vi "FT10xx系列_Coincidence_sample_1.0.3.vi"() -> ()   [LabVIEW 2017]
uses:
  National Instruments/LabVIEW 2017/user.lib/smncsftmt/smncsftmt.lvlib
panel:
  in  "通道选择":i32=1 min=1 max=8
  in  "C18 16":bool
  in  "C17 16":bool
  in  "C16 16":bool
  in  "C15 16":bool
  in  "C14 16":bool
  in  "C13 16":bool
  in  "C12 16":bool=TRUE
  in  "C11 16":bool=TRUE
  in  "窗口宽度(ns)":dbl=1000.0
  in  "停止":bool
  out "error out":errorcluster
  out "通道计数":u64
  out "符合计数":u32
  in  "统计时间(s)":dbl=1.0
  in  "保存路径":path=path "D:/siminics"
  out "已连接？":bool
  # "FT10XX系列符合模式"
  # "选择通道"
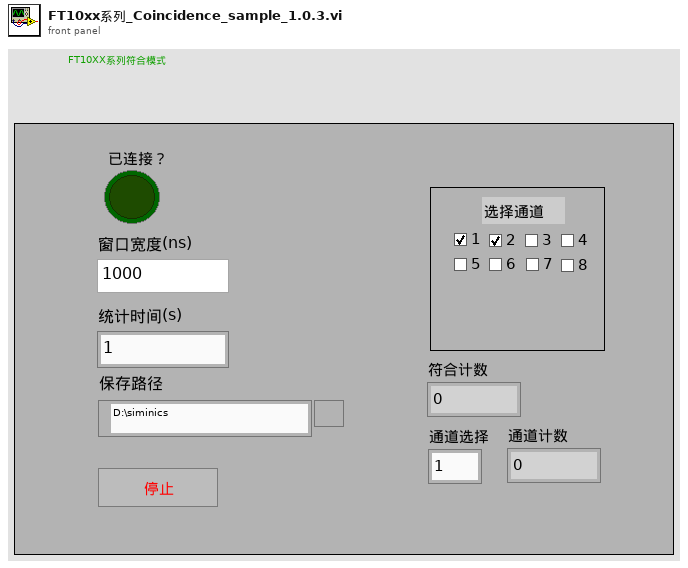
[diagram p1: front panel]
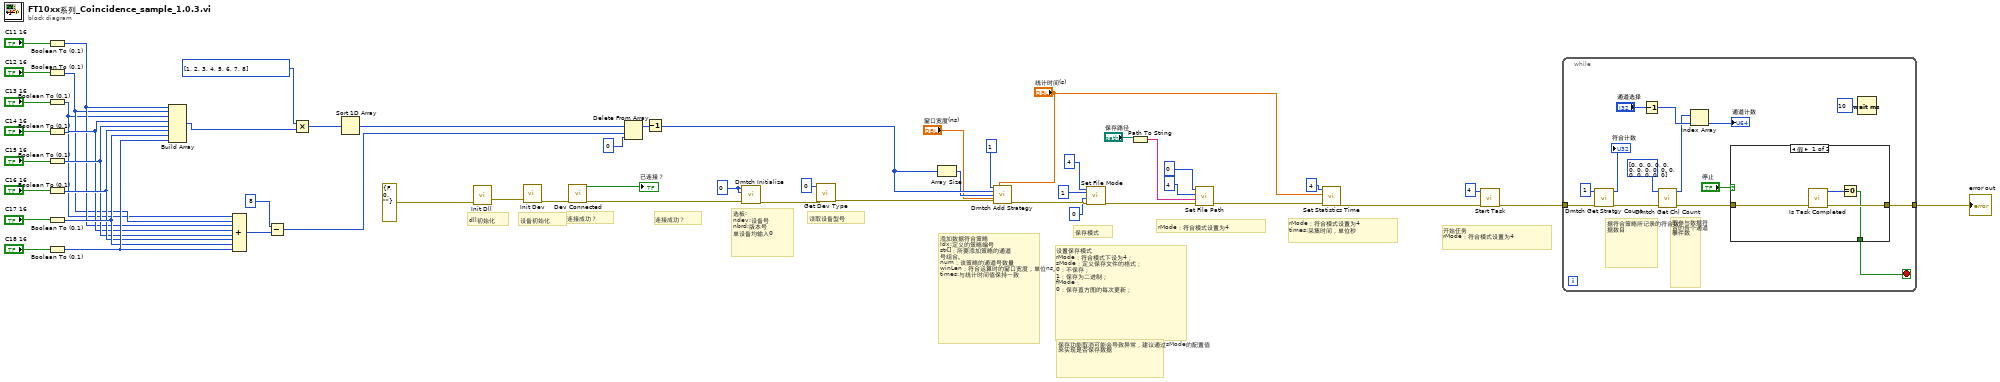
[diagram p0: block diagram]
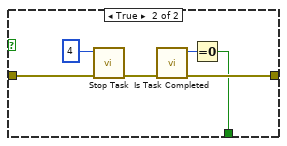
[diagram p2: hidden frame]
diagram:
  w17 = 0
  # "连接成功？"
  # "设备初始化"
  # "dll初始化"
  # "读取设备型号"
  # "开始任务\nrMode：符合模式设置为4"
  # "连接成功？"
  # "保存模式"
  # "保存功能取消可能会导致异常，建议通过sMode的配置值来实现是否保存数据"
  # "设置保存模式\nrMode：符合模式下设为4；\nsMode：定义保存文件的格式；\n0：不保存；\n1：保存为二进制；\nfMode：\n0：保存直方图的每次更新；"
  # "添加数据符合策略\nIdx:定义的策略编号\nstr[]：所要添加策略的通道\n号组合。\nnum：该策略的通道号数量 \nwinLen：符合运算时的窗口宽度，单位ns。  \ntimes:与统计时间值保持一致"
  # "选板:\nndev:设备号\nnbrd:版本号\n单设备均输入0"
  # "rMode：符合模式设置为4"
  # "rMode：符合模式设置为4\ntimes:采集时间，单位秒"
  n1 = Boolean To (0,1)(Boolean="C11 16") -> (0, 1=w26:i16)
  n2 = Boolean To (0,1)(Boolean="C12 16") -> (0, 1=w25:i16)
  n3 = Boolean To (0,1)(Boolean="C13 16") -> (0, 1=w24:i16)
  n4 = Boolean To (0,1)(Boolean="C14 16") -> (0, 1=w27:i16)
  n5 = Boolean To (0,1)(Boolean="C15 16") -> (0, 1=w28:i16)
  n6 = Boolean To (0,1)(Boolean="C16 16") -> (0, 1=w29:i16)
  n7 = Boolean To (0,1)(Boolean="C17 16") -> (0, 1=w30:i16)
  n8 = Boolean To (0,1)(Boolean="C18 16") -> (0, 1=w31:i16)
  n9 = Build Array(w26, w25, w24, w27, w28, w29, w30, w31) -> (w16:i16[])
  n10 = Compound Arithmetic op=ADD(w24, w25, w26, w27, w28, w29, w30, w31) -> (w19:i16)
  n11 = Subtract(x=u16 8, y=w19) -> (x-y=w23:u16)
  n12 = Multiply(x=i32[] [1, 2, 3, 4, 5, 6, 7, 8], y=w16) -> (x*y=w33:i32[])
  n13 = Sort 1D Array(array=w33) -> (sorted array=w36:i32[])
  n14 = call "Init Dll.vi"("error in (no error)"=errorcluster {"status"=FALSE, "code"=0, "source"=""}) -> ("error out"=w9:errorcluster)  [unwired: 9 in, 1 out]
  n15 = call "Init Dev.vi"("error in (no error)"=w9) -> ("error out"=w8:errorcluster)  [unwired: 9 in, 1 out]
  n16 = call "Dev Connected.vi"("error in (no error)"=w8) -> ("error out"=w7:errorcluster, "function return"=→"已连接？":bool)  [unwired: 9 in]
  n17 = Delete From Array(array=w36, length=w23, index=0 ("索引")) -> (array with subset deleted=w34:i32[])  [unwired: 1 out]
  n18 = Decrement(x=w34) -> (x-1=w15:i32[])
  n19 = call "Dmtch Initialize.vi"("error in (no error)"=w7, "nBoard"=w17, "nDevId"=w17) -> ("error out"=w12:errorcluster)  [unwired: 7 in, 1 out]
  n20 = call "Get Dev Type.vi"("error in (no error)"=w12, "nDevId"=0 ("devId")) -> ("error out"=w11:errorcluster)  [unwired: 7 in, 2 out]
  n21 = Array Size(array=w15) -> (size(s)=w13:i32)
  n22 = call "Dmtch Add Strategy.vi"("nIndex"=1 ("idx"), "times"="统计时间(s)", "nStr"=w15, "nNum"=w13, "nWinLen"="窗口宽度(ns)", "error in (no error)"=w11) -> ("error out"=w48:errorcluster)  [unwired: 7 in, 2 out]
  n23 = call "Set File Mode.vi"("error in (no error)"=w48, "nFilterMode"=0 ("fMode"), "nSaveMode"=1, "nRunMode"=4 ("rMode")) -> ("error out"=w49:errorcluster)  [unwired: 6 in, 1 out]
  n24 = Path To String(path="保存路径") -> (string=w51:string)
  n25 = call "Set File Path.vi"("error in (no error)"=w49, "strFilePath"=w51, "nRunMode"=4 ("rMode"), "nDevId"=0 ("nRunMode")) -> ("error out"=w54:errorcluster)  [unwired: 6 in, 1 out]
  n26 = call "Set Statistics Time.vi"("error in (no error)"=w54, "Times"="统计时间(s)", "nRunMode"=4 ("rMode")) -> ("error out"=w22:errorcluster)  [unwired: 7 in, 1 out]
  n27 = call "Start Task.vi"("error in (no error)"=w22, "nRunMode"=4 ("rMode")) -> ("error out"=w21:errorcluster)  [unwired: 8 in, 1 out]
  n28 = while {
    tunnel: w21 -> [w68]
    tunnel: [w62] -> w3
    stop <- w61 stop-if-true
    # "取参与数据符合的各个通道事件数"
    # "据符合策略所记录的符合数据数目"
    n29 = call "Dmtch Get Stratgy Count.vi"("error in (no error)"=w68, "nIndex"=1 ("idx")) -> ("error out"=w65:errorcluster, "function return"=→"符合计数":u32)  [unwired: 8 in]
    n30 = Decrement(x="通道选择") -> (x-1=w59:i32)
    n31 = call "Dmtch Get Chl Count.vi"("error in (no error)"=w65, "chlCnt"=u64[] [0, 0, 0, 0, 0, 0, 0, 0, 0, 0, 0, 0, 0, 0, 0, 0]) -> ("error out"=w64:errorcluster, "chlCnt 2"=w56:u64[])  [unwired: 7 in, 1 out]
    n32 = Index Array(array=w56, index=w59) -> (element=→"通道计数":u64)
    n33 = case shown="假" "停止" {
      tunnel: w64 -> [w71 w77]
      tunnel: [w72 w75] -> w62
      tunnel: [w69 w73] -> w61
      frame False {
        n34 = call "Is Task Completed.vi"("error in (no error)"=w71) -> ("error out"=w72:errorcluster, "function return"=w70:i32)  [unwired: 9 in]
        n35 = Equal To 0?(x=w70) -> (x = 0?=w69:bool)
      }
      frame True {
        n36 = call "Stop Task.vi"("error in (no error)"=w77, "nRunMode"=4 ("rMode")) -> ("error out"=w76:errorcluster)  [unwired: 8 in, 1 out]
        n37 = call "Is Task Completed.vi"("error in (no error)"=w76) -> ("error out"=w75:errorcluster, "function return"=w74:i32)  [unwired: 9 in]
        n38 = Equal To 0?(x=w74) -> (x = 0?=w73:bool)
      }
    }
    n39 = Wait (ms)(milliseconds to wait=u32 10 ("等待时间（毫秒）")) -> ()  [unwired: 1 out]
  }
  "error out" <- w3
